vi "Message.vi"(8 "error in (no error)":errorcluster, 11 "Node Ptr":T2 format="%.0x") -> (0 "error out":errorcluster)   [LabVIEW 2020, in "Instrument Addon System Explorer.lvlib"]
uses:
  Instrument Addon System Explorer.lvlib
  <vilib>/NI VeriStand/Custom Device API/Custom Device API.lvlib
  Addon Shared/Instrument Addon Shared.lvlib
  Addon Shared/Types/FG Control.ctl
  <vilib>/NI VeriStand/Custom Device API/Custom Device Item Ref.ctl
  Addon Shared/Types/Message Generation Type.ctl
panel:
  in  "Type":string(combo)
  in  "Include Protection":bool caption="Include Protection?"
  in  "Period":dbl=1.0 caption="Period (sec)" format="%#_p"
  in  "Generation Type":T1
  in  "Header 2":cluster{"Section Name":string}={"Section Name"="Generation Settings"}
  in  "SHDocVw.IWebBrowser":refnum<k7>(container)
  in  "Header":cluster{"Section Name":string}={"Section Name"="Message Settings"}
  in  "Description":string
  in  "Name":string
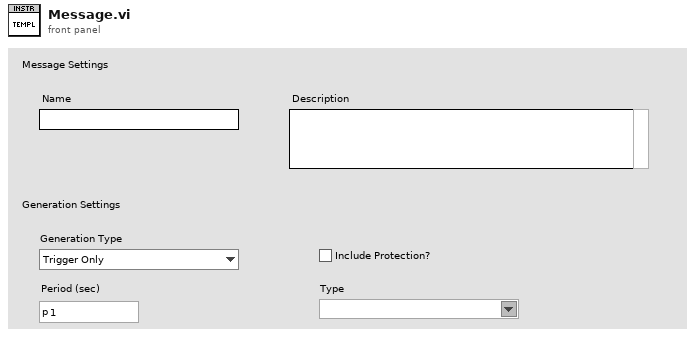
[diagram p1: front panel]
types:
  T1 = typedef "Instrument Addon Shared.lvlib/Message Generation Type.ctl" = enum16{"Trigger Only", "Periodic & Trigger", "Value Change & Trigger"}
  T2 = typedef "Custom Device API.lvlib/Custom Device Item Ref.ctl" = u64
  T3 = typedef "Instrument Addon Shared.lvlib/FG Control.ctl" = enum16{"Get", "Set"}
  T4 = typedef "Instrument Addon Shared.lvlib/Message Parameters.ctl" = cluster{"Generation Type":T1, "Period":dbl, "Include Protection":bool, "Type":string}
  T5 = typedef "Custom Device API.lvlib/Custom Device Item Info.ctl" = cluster{"Name":string, "Is Channel":bool, "GUID":string, "Is Waveform":bool}
  T6 = typedef "Custom Device API.lvlib/Custom Device Commands.ctl" = enum16{"Default", "Item renamed", "Shutdown", "Dynamic button pressed"}
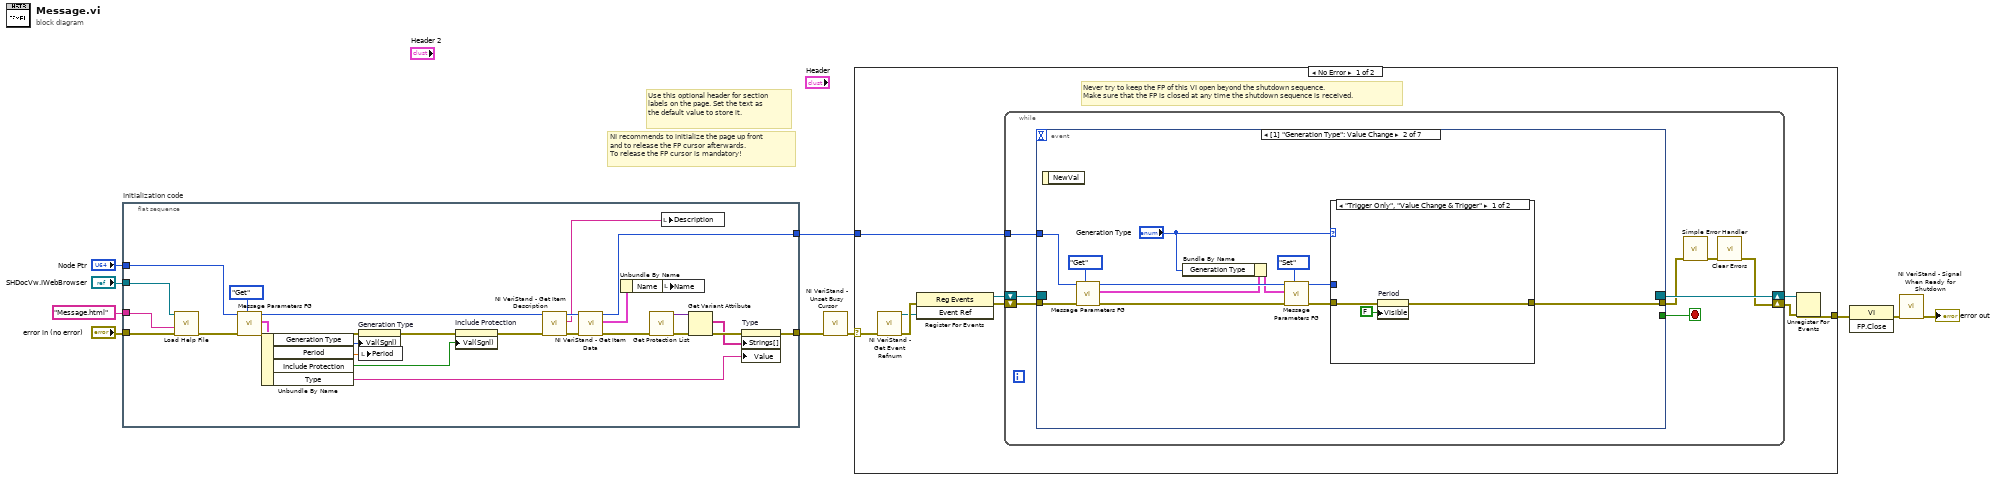
[diagram p0: block diagram]
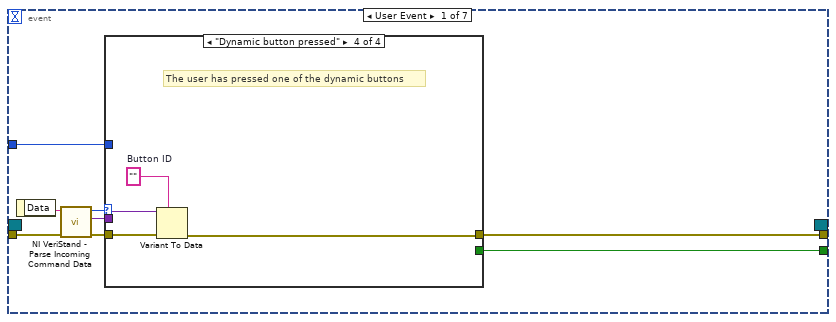
[diagram p2: hidden frame]
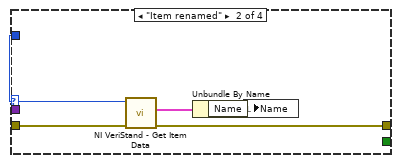
[diagram p4: hidden frame]
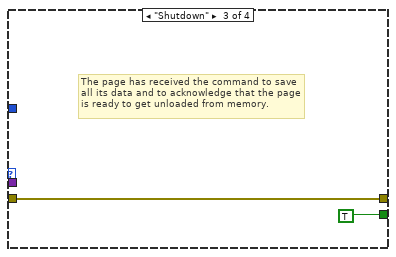
[diagram p5: hidden frame]
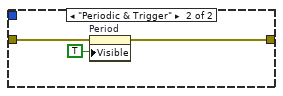
[diagram p6: hidden frame]
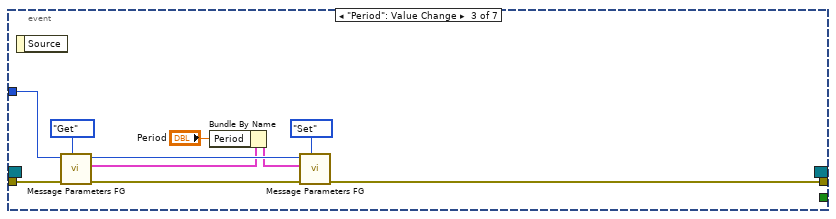
[diagram p7: hidden frame]
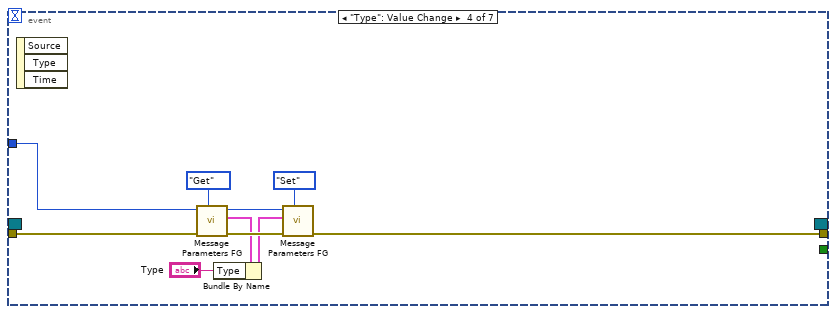
[diagram p8: hidden frame]
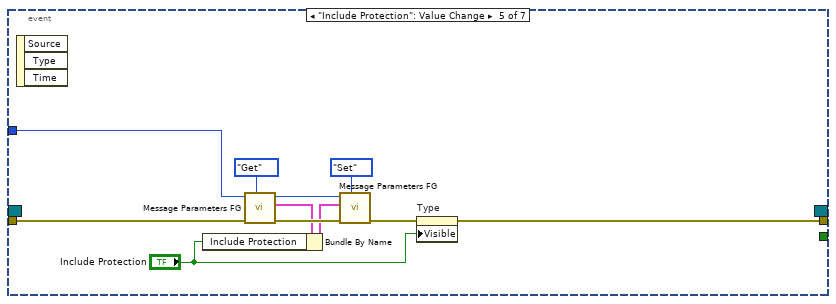
[diagram p9: hidden frame]
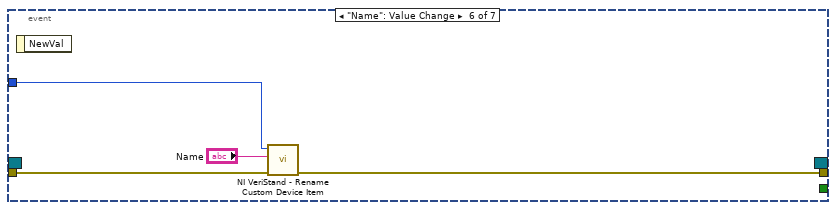
[diagram p10: hidden frame]
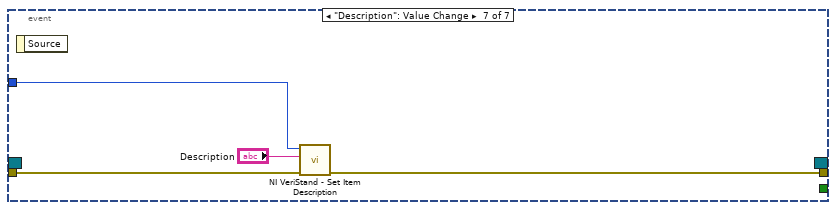
[diagram p11: hidden frame]
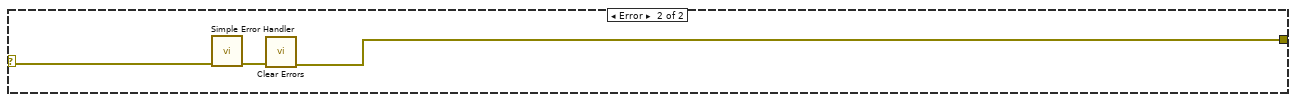
[diagram p12: hidden frame]
diagram:
  # "Use this optional header for section labels on the page. Set the text as the default value to store it."
  # "NI recommends to initialize the page up front\nand to release the FP cursor afterwards.\nTo release the FP cursor is mandatory!"
  n1 = flat-sequence "Initialization code" {
    tunnel: "error in (no error)" -> [w31]
    tunnel: "Node Ptr" -> [w26]
    tunnel: [w12] -> w6
    tunnel: [w37] -> w3
    tunnel: "SHDocVw.IWebBrowser" -> [w30]
    tunnel: "Message.html" ("HTML File") -> [w29]
    frame #0 {
      n2 = call "Load Help File.vi"("error in (no error)"=w31, "HTML File to Load"=w29, "SHDocVw.IWebBrowser2"=w30) -> ("error out"=w27:errorcluster)  [unwired: 8 in]
      n3 = call "Message Parameters FG.vi"("Action"=FG_Control."Get", "error in (no error)"=w27, "Item Ref in"=w26) -> ("error out"=w24:errorcluster, "Message Settings out"=w23:T4, "Item Ref out"=w25:T2)  [unwired: 6 in]
      n4 = Unbundle By Name(w23) -> ("Generation Type"=w22:T1, "Period"=w21:dbl, "Include Protection"=w19:bool, "Type"=w11:string)
      n5 = property on="Generation Type" class="Enum (strict)"(error in=w24, "Val(Sgnl)"=w22) -> (error out=w20:errorcluster)  [unwired: 1 in, 1 out]
      n6 = local write "Period"(w21) -> ()
      n7 = property on="Include Protection" class="Bool (strict)"(error in=w20, "Val(Sgnl)"=w19) -> (error out=w14:errorcluster)  [unwired: 1 in, 1 out]
      n8 = call <vilib>:"NI VeriStand - Get Item Description.vi"("error in (no error)"=w14, "Item Ref in"=w25) -> ("error out"=w34:errorcluster, "Description"=w35:string, "Item Ref out"=w36:T2)  [unwired: 7 out]
      n9 = call <vilib>:"NI VeriStand - Get Item Data.vi"("error in (no error)"=w34, "Item Ref in"=w36) -> ("error out"=w13:errorcluster, "Item Info"=w33:T5, "Item Ref out"=w37:T2)  [unwired: 7 out]
      n10 = Unbundle By Name(w33) -> ("Name"=w32:string)
      n11 = call "Get Protection List.vi"("error in (no error)"=w13) -> ("error out"=w18:errorcluster, "Class Lookup"=w16:variant)  [unwired: 9 in]
      n12 = local write "Description"(w35) -> ()
      n13 = local write "Name"(w32) -> ()
      n14 = Get Variant Attribute(Variant=w16, error in=w18) -> (names=w15:string[], error out=w17:errorcluster)  [unwired: 2 in, 2 out]
      n15 = property on="Type" class="CmbBox"(error in=w17, "Strings[]"=w15, "Value"=w11) -> (error out=w12:errorcluster)  [unwired: 1 in, 1 out]
    }
  }
  n16 = call <vilib>:"NI VeriStand - Unset Busy Cursor.vi"("error in (no error)"=w6) -> ("error out"=w5:errorcluster)  [unwired: 10 out]
  n17 = case shown="No Error" w5 {
    selector: w5 -> [w38 w134]
    tunnel: [w43 w132] -> w10
    tunnel: w3 -> [w39 _]
    frame No Error {
      # "Never try to keep the FP of this VI open beyond the shutdown sequence.\nMake sure that the FP is closed at any time the shutdown sequence is received."
      n18 = call <vilib>:"NI VeriStand - Get Event Refnum.vi"("error in (no error)"=w38) -> ("error out"=w46:errorcluster, "Event Ref"=w42:refnum<user-event>)  [unwired: 9 out]
      n19 = register-events(error in=w46, w42) -> (reference out=w40:refnum<event-registration>, error out=w41:errorcluster)  [unwired: 1 in]
      n20 = while {
        tunnel: w39 -> [w50]
        shift-right: [w47] -> w44
        shift-left: w41 -> [w53]
        shift-right: [w54] -> w45
        shift-left: w40 -> [w52]
        stop <- w51 stop-if-true
        n21 = event shown="[1] \"Generation Type\": Value Change" {
          selector: w52 -> [_ _ _ _ _ _ _]
          dyn-events: [_ _ _ _ _ _ _] -> w54
          timeout: _ -> [_ _ _ _ _ _ _]
          tunnel: w53 -> [w62 w86 w102 w112 w123 w127 w130]
          tunnel: [w58 _ _ _ _ _ _] -> w51
          tunnel: [w57 w77 w94 w104 w113 w126 w129] -> w49
          tunnel: w50 -> [w56 w85 w101 w111 w122 w125 w131]
          event User Event {
            n22 = event-data() -> ("Data"=w61:string)  [unwired: 1 out]
            n23 = call <vilib>:"NI VeriStand - Parse Incoming Command Data.vi"("error in (no error)"=w62, "Incoming data"=w61) -> ("error out"=w60:errorcluster, "Outgoing data"=w55:variant, "Action"=w59:T6)  [unwired: 7 out]
            n24 = case shown="\"Dynamic button pressed\"" w59 {
              tunnel: w60 -> [w63 w68 w69 w74]
              tunnel: [_ _ TRUE _] -> w58
              tunnel: [w63 w65 w69 w71] -> w57
              tunnel: w56 -> [_ w67 _ _]
              tunnel: w55 -> [_ _ _ w73]
              frame "Default", Default {
              }
              frame "Item renamed" {
                n25 = call <vilib>:"NI VeriStand - Get Item Data.vi"("error in (no error)"=w68, "Item Ref in"=w67) -> ("error out"=w65:errorcluster, "Item Info"=w66:T5)  [unwired: 8 out]
                n26 = Unbundle By Name(w66) -> ("Name"=w64:string)
                n27 = local write "Name"(w64) -> ()
              }
              frame "Shutdown" {
                # "The page has received the command to save all its data and to acknowledge that the page is ready to get unloaded from memory."
              }
              frame "Dynamic button pressed" {
                w72 = ""  # Button ID
                # "The user has pressed one of the dynamic buttons"
                n28 = Variant To Data(error in=w74, type=w72, Variant=w73) -> (error out=w71:errorcluster)  [unwired: 1 out]
              }
            }
          }
          event Value Change {
            n29 = event-data() -> ()  [unwired: 2 out]
            n30 = call "Message Parameters FG.vi"("Action"=FG_Control."Get", "error in (no error)"=w86, "Item Ref in"=w85) -> ("error out"=w84:errorcluster, "Message Settings out"=w81:T4, "Item Ref out"=w83:T2)  [unwired: 6 in]
            n31 = Bundle By Name(cluster=w81, "Generation Type"="Generation Type") -> (w80:T4)
            n32 = call "Message Parameters FG.vi"("Action"=FG_Control."Set", "error in (no error)"=w84, "Message Settings"=w80, "Item Ref in"=w83) -> ("error out"=w78:errorcluster, "Item Ref out"=w75:T2)  [unwired: 5 in, 1 out]
            n33 = case shown="\"Trigger Only\", \"Value Change & Trigger\"" "Generation Type" {
              tunnel: w78 -> [w88 w92]
              tunnel: [w87 w90] -> w77
              tunnel: w75 -> [_ _]
              frame "Trigger Only", "Value Change & Trigger" {
                n34 = property on="Period" class="DigNum (strict)"(error in=w88, "Visible"=FALSE) -> (error out=w87:errorcluster)  [unwired: 1 in, 1 out]
              }
              frame "Periodic & Trigger" {
                n35 = property on="Period" class="DigNum (strict)"(error in=w92, "Visible"=TRUE) -> (error out=w90:errorcluster)  [unwired: 1 in, 1 out]
              }
            }
          }
          event "Period": Value Change {
            n36 = event-data() -> ()  [unwired: 2 out]
            n37 = call "Message Parameters FG.vi"("Action"=FG_Control."Get", "error in (no error)"=w102, "Item Ref in"=w101) -> ("error out"=w100:errorcluster, "Message Settings out"=w97:T4, "Item Ref out"=w99:T2)  [unwired: 6 in]
            n38 = Bundle By Name(cluster=w97, "Period"="Period") -> (w96:T4)
            n39 = call "Message Parameters FG.vi"("Action"=FG_Control."Set", "error in (no error)"=w100, "Message Settings"=w96, "Item Ref in"=w99) -> ("error out"=w94:errorcluster)  [unwired: 5 in, 2 out]
          }
          event "Type": Value Change {
            n40 = event-data() -> ()  [unwired: 4 out]
            n41 = call "Message Parameters FG.vi"("Action"=FG_Control."Get", "error in (no error)"=w112, "Item Ref in"=w111) -> ("error out"=w110:errorcluster, "Message Settings out"=w107:T4, "Item Ref out"=w109:T2)  [unwired: 6 in]
            n42 = Bundle By Name(cluster=w107, "Type"="Type") -> (w106:T4)
            n43 = call "Message Parameters FG.vi"("Action"=FG_Control."Set", "error in (no error)"=w110, "Message Settings"=w106, "Item Ref in"=w109) -> ("error out"=w104:errorcluster)  [unwired: 5 in, 2 out]
          }
          event "Include Protection": Value Change {
            n44 = event-data() -> ()  [unwired: 4 out]
            n45 = call "Message Parameters FG.vi"("Action"=FG_Control."Get", "error in (no error)"=w123, "Item Ref in"=w122) -> ("error out"=w121:errorcluster, "Message Settings out"=w118:T4, "Item Ref out"=w120:T2)  [unwired: 6 in]
            n46 = Bundle By Name(cluster=w118, "Include Protection"="Include Protection") -> (w117:T4)
            n47 = call "Message Parameters FG.vi"("Action"=FG_Control."Set", "error in (no error)"=w121, "Message Settings"=w117, "Item Ref in"=w120) -> ("error out"=w114:errorcluster)  [unwired: 5 in, 2 out]
            n48 = property on="Type" class="CmbBox"(error in=w114, "Visible"="Include Protection") -> (error out=w113:errorcluster)  [unwired: 1 in, 1 out]
          }
          event "Name": Value Change {
            n49 = event-data() -> ()  [unwired: 2 out]
            n50 = call <vilib>:"NI VeriStand - Rename Custom Device Item.vi"("error in (no error)"=w127, "New Name"="Name", "Item Ref in"=w125) -> ("error out"=w126:errorcluster)  [unwired: 1 in, 7 out]
          }
          event "Description": Value Change {
            n51 = event-data() -> ()  [unwired: 2 out]
            n52 = call <vilib>:"NI VeriStand - Set Item Description.vi"("error in (no error)"=w130, "Description"="Description", "Item Ref in"=w131) -> ("error out"=w129:errorcluster)  [unwired: 8 out]
          }
        }
        n53 = call <vilib>:"Simple Error Handler.vi"("error in (no error)"=w49) -> ("error out"=w48:errorcluster)  [unwired: 1 in, 7 out]
        n54 = call <vilib>:"Clear Errors.vi"("error in (no error)"=w48) -> ("error out"=w47:errorcluster)  [unwired: 1 in, 5 out]
      }
      n55 = Unregister For Events(event registration refnum=w45, error in=w44) -> (error out=w43:errorcluster)
    }
    frame Error {
      n56 = call <vilib>:"Simple Error Handler.vi"("error in (no error)"=w134) -> ("error out"=w133:errorcluster)  [unwired: 1 in, 7 out]
      n57 = call <vilib>:"Clear Errors.vi"("error in (no error)"=w133) -> ("error out"=w132:errorcluster)  [unwired: 1 in, 5 out]
    }
  }
  n58 = invoke class="VI" method="FP.Close"(error in=w10) -> (error out=w9:errorcluster)  [unwired: 2 in, 2 out]
  n59 = call <vilib>:"NI VeriStand - Signal When Ready for Shutdown.vi"("error in (no error)"=w9) -> ("error out"=→"error out":errorcluster)  [unwired: 10 out]
